vi "Parse Results (all).vi"(6 "Type":T1, 8 "error in (no error)":errorcluster, 11 "Results (Dictionary)":cluster{"key":string, "value":dbl}[](array[cluster])) -> (0 "error out":errorcluster, 1 "Label":string[](array[string]), 2 "Data":dbl[](array[numeric]), 3 "Results (Dictionary)":cluster{"key":string, "value":dbl}[](array[cluster]))   [LabVIEW 2019, in "Instrument.Lockin.lvlib" / "Instrument.Lockin.lvclass"]
doc: "This method will search the <b>Results Dictionary</b> for the data specified by <b>Datatype</b> (X, Y, R, Theta, mean).\n\n<b>Data</b> is an array of clusters, of which each element is an array of the matched datatype."
uses:
  Instrument.Lockin.lvclass
  Typedefs/Results Type--Enum.ctl
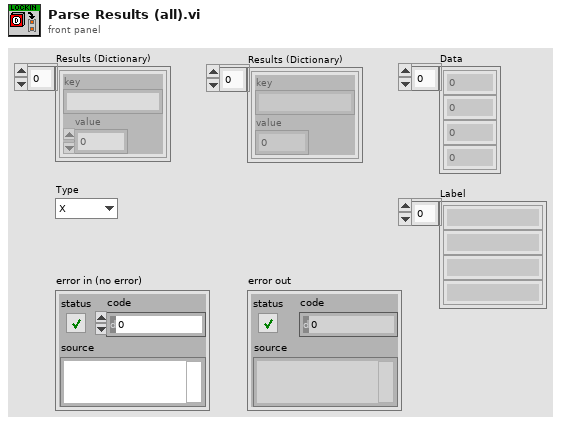
[diagram p1: front panel]
types:
  T1 = typedef "Instrument.Lockin.lvlib/Instrument.Lockin.lvclass/Results Type--Enum.ctl" = enum16{"X", "Y", "R", "Theta", "Mean"}
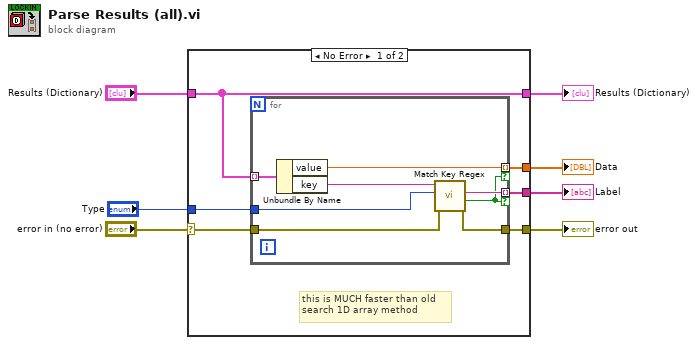
[diagram p0: block diagram]
diagram:
  n1 = case shown="No Error" "error in (no error)" {
    selector: "error in (no error)" -> [w11 w22]
    tunnel: "Type" -> [w12 _]
    tunnel: "Results (Dictionary)" -> [w13 w23]
    tunnel: [w10 _] -> w5
    tunnel: [w9 w22] -> w2
    tunnel: [w13 w23] -> w4
    tunnel: [w8 _] -> w1
    frame No Error {
      # "this is MUCH faster than old\nsearch 1D array method"
      n2 = for {
        tunnel: [w14] -> w8 mode=indexing if=w18
        tunnel: w13 -> [w21] mode=indexing
        tunnel: w12 -> [w15]
        tunnel: w11 -> [w17]
        tunnel: [w19] -> w10 mode=indexing if=w18
        tunnel: [w16] -> w9
        n3 = Unbundle By Name(w21) -> ("value"=w14:dbl, "key"=w20:string)
        n4 = call "Match Key Regex.vi"("error in"=w17, "Datatype"=w15, "key in"=w20) -> ("error out"=w16:errorcluster, "Datatype Found?"=w18:bool, "Label out"=w19:string)  [unwired: 5 in, 1 out]
      }
    }
    frame Error {
    }
  }
  "Data" <- w1
  "Results (Dictionary)" <- w4
  "Label" <- w5
  "error out" <- w2
